vi "ZM-TST-routing.vi"() -> (0 "error out":errorcluster, 3 "Pass":bool)   [LabVIEW 2020, in "ZM-TST-tests.lvlib"]
doc: "T7, test of the root's routing: calls ZM-CI-handlePackage on a default root with test packages to Hardware, Unknown and Communication, and checks in the error log that the first two are dropped and the third is not. Pass = AND of the four checks. Side effect: two dropped lines in the error log."
uses:
  ZM-TST-tests.lvlib
  actors/ZM-ROOT-root/ZM-ROOT-root/ZM-ROOT-root.lvclass
  common/ZM-PC-packages/ZM-PC-TP-test_package/ZM-PC-TP-test_package.lvclass
  common/ZM-PC-packages/ZM-PC-package/ZM-PC-package.lvclass
panel:
  out "no_error_ok":bool
  out "communication_not_dropped_ok":bool
  out "unknown_dropped_ok":bool
  out "hardware_dropped_ok":bool
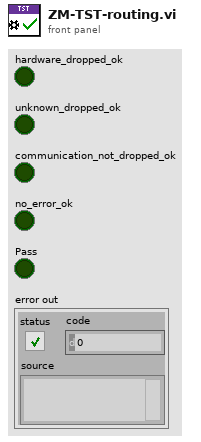
[diagram p1: front panel]
types:
  T1 = enum16{"Unknown", "Root", "Hardware", "Communication"}
  T2 = cluster{"temperature_c":dbl, "sample_index":i32, "duty_percent":u8, "sensor_ok":bool, "status":string}
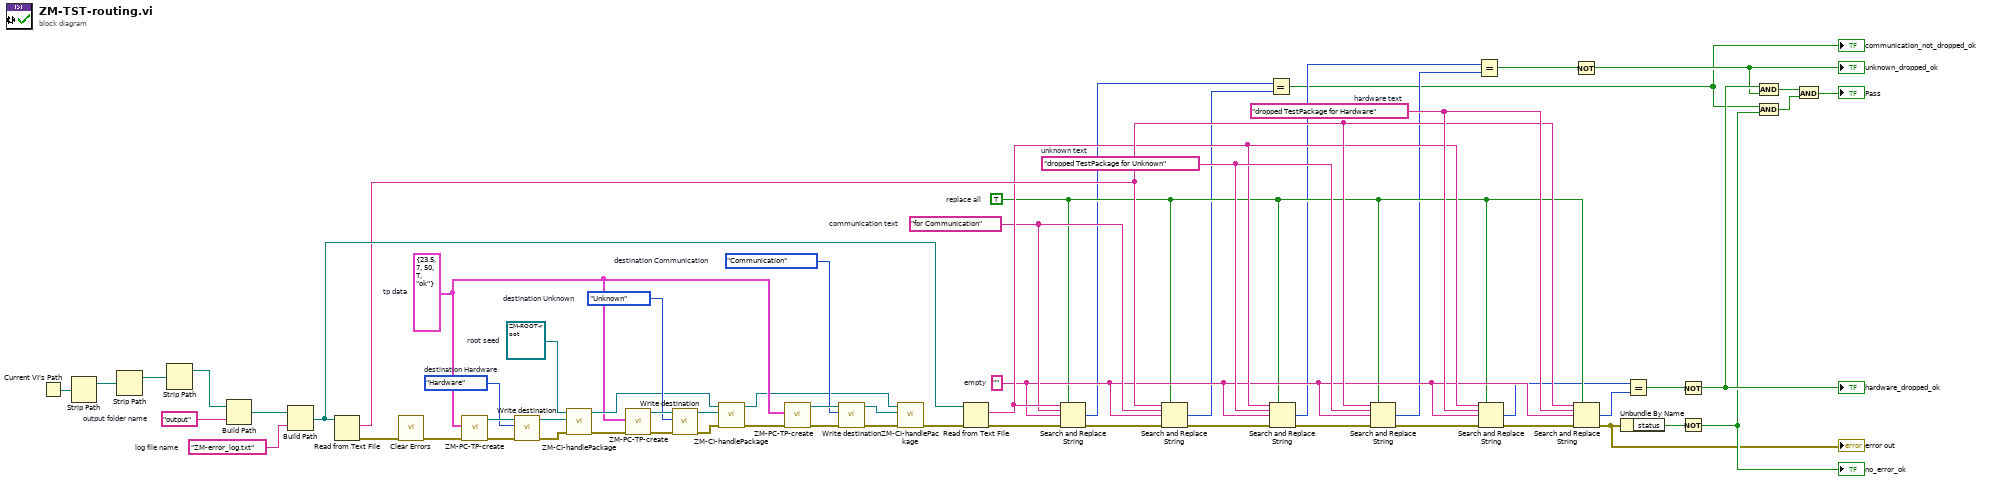
[diagram p0: block diagram]
diagram:
  w24 = TRUE  # replace all
  w25 = ""  # empty
  w26 = "for Communication"  # communication text
  w29 = "dropped TestPackage for Unknown"  # unknown text
  w30 = "dropped TestPackage for Hardware"  # hardware text
  w56 = "ZM-error_log.txt"  # log file name
  w58 = "output"  # output folder name
  w36 = T1."Communication"  # destination Communication
  w44 = T1."Unknown"  # destination Unknown
  w51 = T1."Hardware"  # destination Hardware
  w40 = T2 {"temperature_c"=23.5, "sample_index"=7, "duty_percent"=50, "sensor_ok"=TRUE, "status"="ok"}  # tp data
  w50 = refnum<class "ZM-ROOT-root.lvclass"> refnum  # root seed
  n1 = Current VI's Path() -> (path=w62:path)
  n2 = Strip Path(path=w62) -> (stripped path=w61:path)  [unwired: 1 out]
  n3 = Strip Path(path=w61) -> (stripped path=w60:path)  [unwired: 1 out]
  n4 = Strip Path(path=w60) -> (stripped path=w59:path)  [unwired: 1 out]
  n5 = Build Path(base path=w59, name or relative path=w58) -> (appended path=w57:path)
  n6 = Build Path(base path=w57, name or relative path=w56) -> (appended path=w32:path)
  n7 = Read from Text File(file (use dialog)=w32) -> (text=w28:string, error out=w55:errorcluster)  [unwired: 3 in, 2 out]
  n8 = call <vilib>:"Clear Errors.vi"("error in (no error)"=w55) -> ("error out"=w54:errorcluster)  [unwired: 5 in, 1 out]
  n9 = call "ZM-PC-TP-create.vi"("error in (no error)"=w54, "data"=w40) -> ("error out"=w53:errorcluster, "package"=w52:refnum<class "ZM-PC-TP-test_package.lvclass">)  [unwired: 8 in]
  n10 = call "Write destination.vi"("error in (no error)"=w53, "ZM-PC-DESTINATION"=w51, "ZM-PC-package in"=w52) -> ("error out"=w48:errorcluster, "ZM-PC-package out"=w49:refnum<class "ZM-PC-TP-test_package.lvclass">)  [unwired: 7 in]
  n11 = call-dynamic "ZM-CI-handlePackage.vi"("error in (no error)"=w48, "package"=w49, "ZM-ROOT-root in"=w50) -> ("error out"=w47:errorcluster, "ZM-ROOT-root out"=w43:refnum<class "ZM-ROOT-root.lvclass">)  [unwired: 7 in]
  n12 = call "ZM-PC-TP-create.vi"("error in (no error)"=w47, "data"=w40) -> ("error out"=w46:errorcluster, "package"=w45:refnum<class "ZM-PC-TP-test_package.lvclass">)  [unwired: 8 in]
  n13 = call "Write destination.vi"("error in (no error)"=w46, "ZM-PC-DESTINATION"=w44, "ZM-PC-package in"=w45) -> ("error out"=w41:errorcluster, "ZM-PC-package out"=w42:refnum<class "ZM-PC-TP-test_package.lvclass">)  [unwired: 7 in]
  n14 = call-dynamic "ZM-CI-handlePackage.vi"("error in (no error)"=w41, "package"=w42, "ZM-ROOT-root in"=w43) -> ("error out"=w39:errorcluster, "ZM-ROOT-root out"=w35:refnum<class "ZM-ROOT-root.lvclass">)  [unwired: 7 in]
  n15 = call "ZM-PC-TP-create.vi"("error in (no error)"=w39, "data"=w40) -> ("error out"=w38:errorcluster, "package"=w37:refnum<class "ZM-PC-TP-test_package.lvclass">)  [unwired: 8 in]
  n16 = call "Write destination.vi"("error in (no error)"=w38, "ZM-PC-DESTINATION"=w36, "ZM-PC-package in"=w37) -> ("error out"=w33:errorcluster, "ZM-PC-package out"=w34:refnum<class "ZM-PC-TP-test_package.lvclass">)  [unwired: 7 in]
  n17 = call-dynamic "ZM-CI-handlePackage.vi"("error in (no error)"=w33, "package"=w34, "ZM-ROOT-root in"=w35) -> ("error out"=w31:errorcluster)  [unwired: 7 in, 1 out]
  n18 = Read from Text File(file (use dialog)=w32, error in=w31) -> (text=w27:string, error out=w7:errorcluster)  [unwired: 2 in, 2 out]
  n19 = Search and Replace String(replace all?=w24, input string=w27, search string=w26, replace string=w25, error in=w7) -> (number of replacements=w17:i32, error out=w6:errorcluster)  [unwired: 3 in, 2 out]
  n20 = Search and Replace String(replace all?=w24, input string=w28, search string=w26, replace string=w25, error in=w6) -> (number of replacements=w16:i32, error out=w5:errorcluster)  [unwired: 3 in, 2 out]
  n21 = Equal?(x=w17, y=w16) -> (x = y?=w10:bool)
  "communication_not_dropped_ok" <- w10
  n22 = Search and Replace String(replace all?=w24, input string=w27, search string=w29, replace string=w25, error in=w5) -> (number of replacements=w20:i32, error out=w4:errorcluster)  [unwired: 3 in, 2 out]
  n23 = Search and Replace String(replace all?=w24, input string=w28, search string=w29, replace string=w25, error in=w4) -> (number of replacements=w19:i32, error out=w3:errorcluster)  [unwired: 3 in, 2 out]
  n24 = Equal?(x=w20, y=w19) -> (x = y?=w18:bool)
  n25 = Search and Replace String(replace all?=w24, input string=w27, search string=w30, replace string=w25, error in=w3) -> (number of replacements=w23:i32, error out=w2:errorcluster)  [unwired: 3 in, 2 out]
  n26 = Not(x=w18) -> (.not. x?=w11:bool)
  "unknown_dropped_ok" <- w11
  n27 = Search and Replace String(replace all?=w24, input string=w28, search string=w30, replace string=w25, error in=w2) -> (number of replacements=w22:i32, error out=w1:errorcluster)  [unwired: 3 in, 2 out]
  "error out" <- w1
  n28 = Unbundle By Name(w1) -> ("status"=w15:bool)
  n29 = Equal?(x=w23, y=w22) -> (x = y?=w21:bool)
  n30 = Not(x=w21) -> (.not. x?=w12:bool)
  "hardware_dropped_ok" <- w12
  n31 = Not(x=w15) -> (.not. x?=w9:bool)
  "no_error_ok" <- w9
  n32 = And(x=w12, y=w11) -> (x .and. y?=w14:bool)
  n33 = And(x=w10, y=w9) -> (x .and. y?=w13:bool)
  n34 = And(x=w14, y=w13) -> (x .and. y?=→"Pass":bool)
